vi "Show Sequence.vi"(8 "error in (no error)":errorcluster, 10 "Sequence":string, 11 "SequenceViewPanel in":refnum<class "SequenceViewPanel.lvclass">) -> (0 "error out":errorcluster, 3 "SequenceViewPanel out":refnum<class "SequenceViewPanel.lvclass">)   [LabVIEW 2020, in "TSnax UI.lvlib" / "SequenceViewPanel.lvclass"]
uses:
  SequenceViewPanel.lvclass
  TSnax/Step Group.ctl
  SequenceViewPanel.lvclass/SequenceViewPanel.ctl
  TSnax/SequenceFile/SequenceFile.lvclass
  TSnax/TSnax.lvlib
  TSnax/Execution/Execution.lvclass
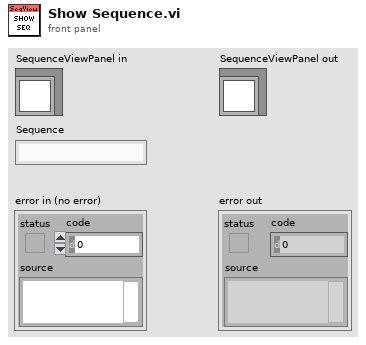
[diagram p1: front panel]
types:
  T1 = typedef "TSnax.lvlib/Step Group.ctl" = enum16{"Setup", "Main", "Cleanup"}
  T2 = typedef "TSnax UI.lvlib/SequenceViewPanel.lvclass/Ref Data.ctl" = cluster{"Insert Line":i32, "SequenceFile":refnum<class "SequenceFile.lvclass">, "Sequence":string, "Trace Marker":i32, "Execution":refnum<class "Execution.lvclass">}
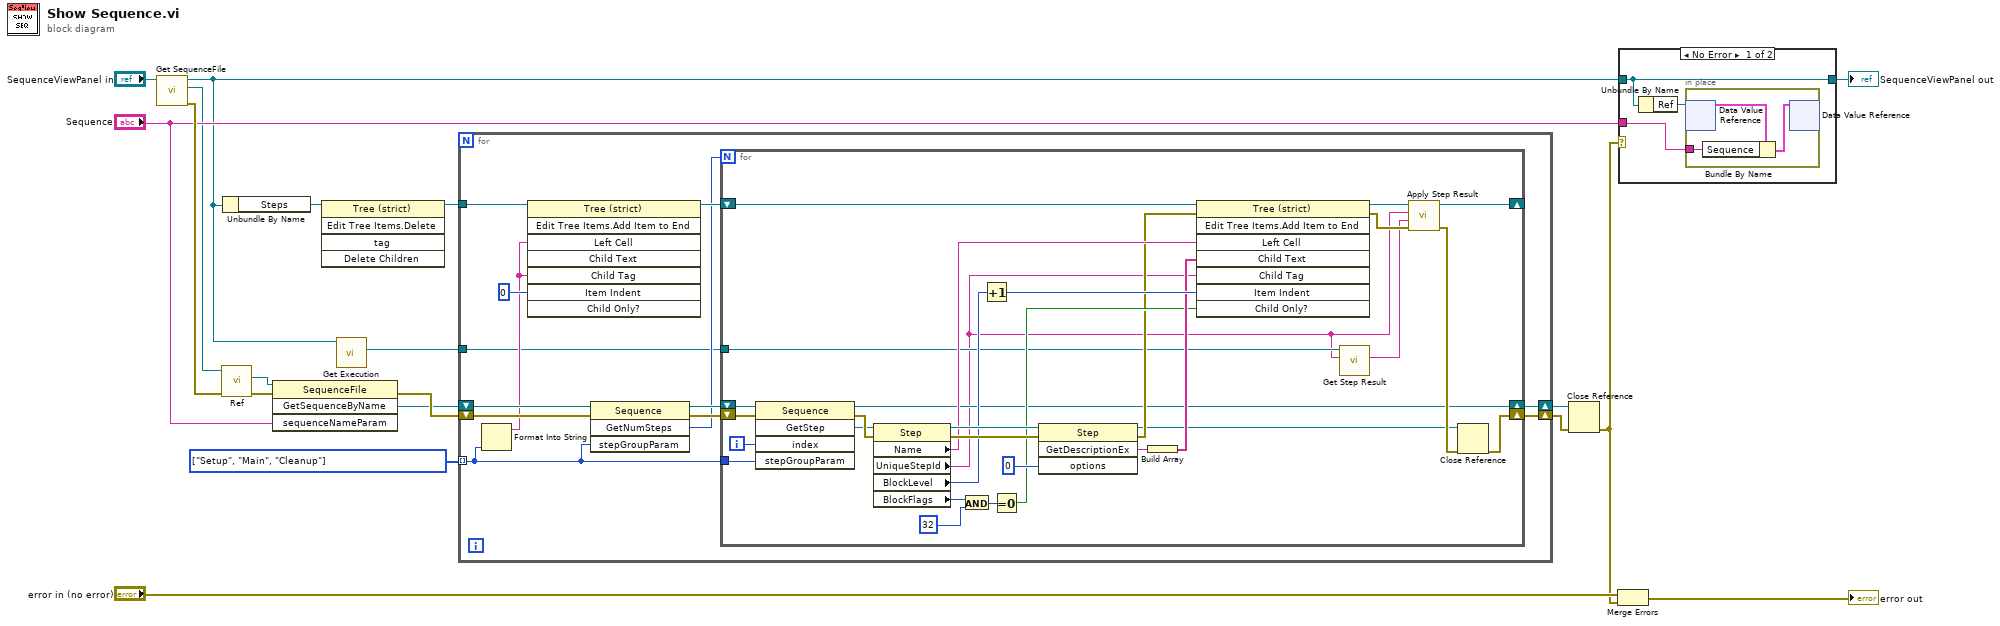
[diagram p0: block diagram]
diagram:
  w12 = T1[] [enum."Setup", enum."Main", enum."Cleanup"] items=["Setup", "Main", "Cleanup"]
  n1 = call "Get SequenceFile.vi"("SequenceViewPanel in"="SequenceViewPanel in") -> ("error out"=w16:errorcluster, "SequenceFile"=w3:refnum<class "SequenceFile.lvclass">, "SequenceViewPanel out"=w2:refnum<class "SequenceViewPanel.lvclass">)  [unwired: 8 in]
  n2 = call "Ref.vi"("error in (no error)"=w16, "SequenceFile in"=w3) -> ("error out"=w14:errorcluster, "Ref"=w15:refnum<k7>)  [unwired: 7 in, 1 out]
  n3 = Unbundle By Name(w2) -> ("Steps"=w11:refnum<vi>)
  n4 = invoke class="SequenceFile" method="GetSequenceByName"(reference=w15, error in=w14, "sequenceNameParam"="Sequence") -> (error out=w19:errorcluster, "GetSequenceByName"=w13:refnum<k7>)  [unwired: 1 in, 2 out]
  n5 = invoke class="Tree (strict)" method="Edit Tree Items.Delete"(reference=w11) -> (reference out=w10:refnum<vi>)  [unwired: 4 in, 4 out]
  n6 = call "Get Execution.vi"("SequenceViewPanel in"=w2) -> ("Execution"=w1:refnum<class "Execution.lvclass">)  [unwired: 8 in, 2 out]
  n7 = for {
    tunnel: w12 -> [w23] mode=indexing
    tunnel: w10 -> [w30]
    shift-right: [w21] -> w8
    shift-left: w19 -> [w32]
    shift-right: [w22] -> w9
    shift-left: w13 -> [w31]
    tunnel: w1 -> [w20]
    n8 = Format Into String(w23) -> (resulting string=w28:string)  [unwired: 3 in, 1 out]
    n9 = invoke class="Tree (strict)" method="Edit Tree Items.Add Item to End"(reference=w30, "Left Cell"=w28, "Child Tag"=w28, "Item Indent"=0 ("New Item Indentation")) -> (reference out=w27:refnum<vi>)  [unwired: 4 in, 7 out]
    n10 = invoke class="Sequence" method="GetNumSteps"(reference=w31, error in=w32, "stepGroupParam"=w23) -> (reference out=w26:refnum<k7>, error out=w25:errorcluster, "GetNumSteps"=w24:i32)  [unwired: 1 in, 1 out]
    n11 = for {
      N: w24 -> [_]
      shift-right: [w36] -> _
      shift-left: w27 -> [w43]
      shift-right: [w41] -> w22
      shift-left: w26 -> [w60]
      shift-right: [w37] -> w21
      shift-left: w25 -> [w59]
      tunnel: w23 -> [w57]
      tunnel: w20 -> [w35]
      i -> [w58]
      n12 = invoke class="Sequence" method="GetStep"(reference=w60, error in=w59, "index"=w58, "stepGroupParam"=w57) -> (reference out=w41:refnum<k7>, error out=w61:errorcluster, "GetStep"=w56:refnum<k7>)  [unwired: 1 in, 2 out]
      n13 = property class="Step"(reference=w56, error in=w61) -> (reference out=w55:refnum<k7>, error out=w54:errorcluster, "Name"=w52:string, "UniqueStepId"=w34:string, "BlockLevel"=w51:i32, "BlockFlags"=w49:i32)
      n14 = And(x=w49, y=32) -> (x .and. y?=w45:i32)
      n15 = Increment(x=w51) -> (x+1=w50:i32)
      n16 = Equal To 0?(x=w45) -> (x = 0?=w44:bool)
      n17 = invoke class="Step" method="GetDescriptionEx"(reference=w55, error in=w54, "options"=0) -> (reference out=w38:refnum<k7>, error out=w42:errorcluster, "GetDescriptionEx"=w47:string)  [unwired: 1 in, 1 out]
      n18 = Build Array(w47) -> (w46:string[])
      n19 = invoke class="Tree (strict)" method="Edit Tree Items.Add Item to End"(reference=w43, error in=w42, "Left Cell"=w52, "Child Text"=w46, "Child Tag"=w34, "Item Indent"=w50, "Child Only?"=w44) -> (reference out=w40:refnum<vi>, error out=w39:errorcluster)  [unwired: 1 in, 6 out]
      n20 = call "Get Step Result.vi"("Step ID"=w34, "Execution in"=w35) -> ("Result Status"=w33:string)  [unwired: 6 in, 3 out]
      n21 = call "Apply Step Result.vi"("error in (no error)"=w39, "ResultStatus"=w33, "UniqueStepId"=w34, "Steps Tree In"=w40) -> ("error out"=w62:errorcluster, "Steps Tree"=w36:refnum<vi>)  [unwired: 6 in]
      n22 = Close Reference(reference=w38, error in (no error)=w62) -> (error out=w37:errorcluster)
    }
  }
  n23 = Close Reference(reference=w9, error in (no error)=w8) -> (error out=w6:errorcluster)
  n24 = Merge Errors("error in (no error)", w6) -> (→"error out":errorcluster)
  n25 = case shown="No Error" w6 {
    tunnel: w2 -> [w64 w69]
    tunnel: [w64 w69] -> w5
    tunnel: "Sequence" -> [w63 _]
    frame No Error {
      n26 = Unbundle By Name(w64) -> ("Ref"=w65:refnum<data-value>)
      n27 = in-place {
        in-place-border: w63 -> [w66]
        n28 = in-place-dvr #1(w65) -> (w68:T2)  [unwired: 1 out]
        n29 = Bundle By Name(cluster=w68, "Sequence"=w66) -> (w67:T2)
        n30 = in-place-dvr #1(w67) -> ()  [unwired: 2 out]
      }
    }
    frame Error {
    }
  }
  "SequenceViewPanel out" <- w5
